vi "Map License Type.vi"(10 "API License":i32, 11 "TSS License In":T1) -> (2 "TSS License":T1, 3 "API License":i32)   [LabVIEW 2020, in "TSS.lvlib" / "Engine.lvclass"]
uses:
  Engine.lvclass
  TS License Type.ctl
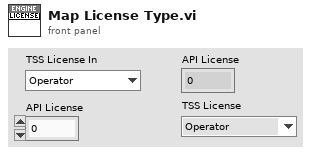
[diagram p1: front panel]
types:
  T1 = typedef "TSS.lvlib/Engine.lvclass/TS License Type.ctl" = enum16{"Operator", "CustomEditor", "SequenceEditor"}
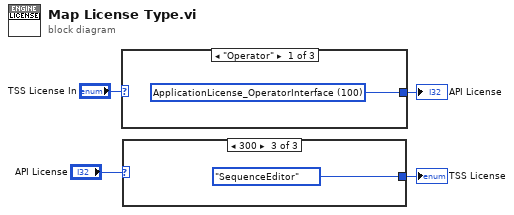
[diagram p0: block diagram]
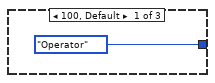
[diagram p2: hidden frame]
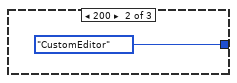
[diagram p3: hidden frame]
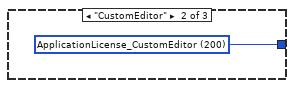
[diagram p4: hidden frame]
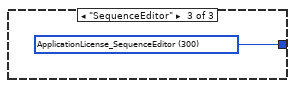
[diagram p5: hidden frame]
diagram:
  n1 = case shown="\"Operator\"" "TSS License In" {
    tunnel: [w5 w6 w7] -> w3
    frame "Operator" {
      w5 = 100 items=["ApplicationLicense_Unspecified"=0, "ApplicationLicense_OperatorInterface"=100, "ApplicationLicense_CustomEditor"=200, "ApplicationLicense_SequenceEditor"=300] ("license")
    }
    frame "CustomEditor" {
      w6 = 200 items=["ApplicationLicense_Unspecified"=0, "ApplicationLicense_OperatorInterface"=100, "ApplicationLicense_CustomEditor"=200, "ApplicationLicense_SequenceEditor"=300] ("license")
    }
    frame "SequenceEditor" {
      w7 = 300 items=["ApplicationLicense_Unspecified"=0, "ApplicationLicense_OperatorInterface"=100, "ApplicationLicense_CustomEditor"=200, "ApplicationLicense_SequenceEditor"=300] ("license")
    }
  }
  "API License" <- w3
  n2 = case shown="300" "API License" {
    tunnel: [TS_License_Type."Operator" ("TSS License") TS_License_Type."CustomEditor" ("TSS License") TS_License_Type."SequenceEditor" ("TSS License")] -> w1
    frame 100, Default {
    }
    frame 200 {
    }
    frame 300 {
    }
  }
  "TSS License" <- w1
